vi "OpenHandle Verify Unwired.vi"(11 "error in":errorcluster) -> (15 "error out":errorcluster)   [LabVIEW 2024]
doc: "Static analysis fixture with verify server unwired and a permanent false guard."
uses:
  <vilib>/httpClient/LabVIEWHTTPClient.lvlib
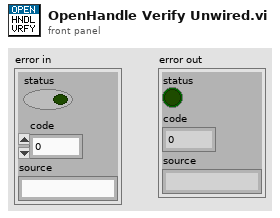
[diagram p1: front panel]
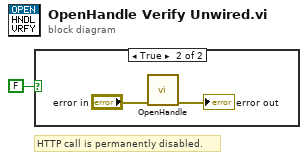
[diagram p0: block diagram]
diagram:
  # "HTTP call is permanently disabled."
  n1 = case shown="True" FALSE ("guard") {
    frame False {
    }
    frame True {
      n2 = call <vilib>:"OpenHandle.vi"("error in (no error)"="error in") -> ("error out"=→"error out":errorcluster)  [unwired: 13 in, 1 out]
    }
  }
